vi "Parse Set Input.vi"(7 "error in (no error)":errorcluster caption="에러 입력(에러 없음)", 9 "JSON string":string, 10 "Instrument Manager 입력":refnum<class "Instrument Manager.lvclass">) -> (0 "error out":errorcluster caption="에러 출력", 1 "Input path":T1, 2 "Set Input Param":T2, 3 "Instrument Manager 출력":refnum<class "Instrument Manager.lvclass">)   [LabVIEW 2023, in "Instrument Manager.lvclass"]
uses:
  Instrument Manager.lvclass
  Param Definition/Set Input Path Param.ctl
  Instrument Manager.lvclass/Instrument Manager.ctl
  Module/CE RF Switch Box/Type Definition/Input path.ctl
  Module/CE RF Switch Box/RF Switch Box.lvlib
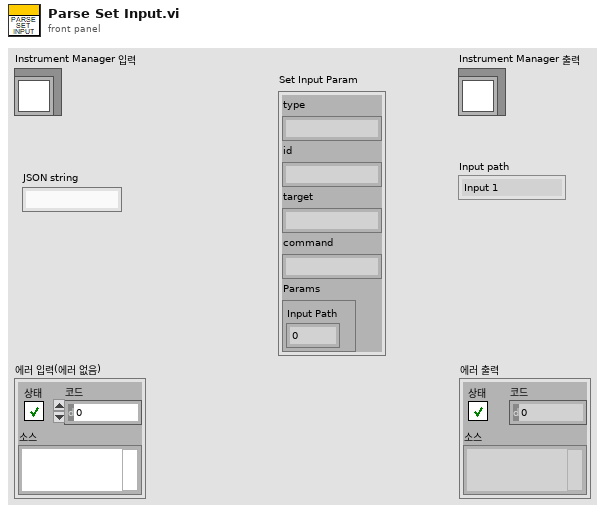
[diagram p1: front panel]
types:
  T1 = typedef "RF Switch Box.lvlib/Input path.ctl" = enum16{"Input 1", "Input 2", "Input 3"}
  T2 = typedef "Instrument Manager.lvclass/Set Input Path Param.ctl" = cluster{"type":string, "id":string, "target":string, "command":string, "Params":cluster{"Input Path":i32}}
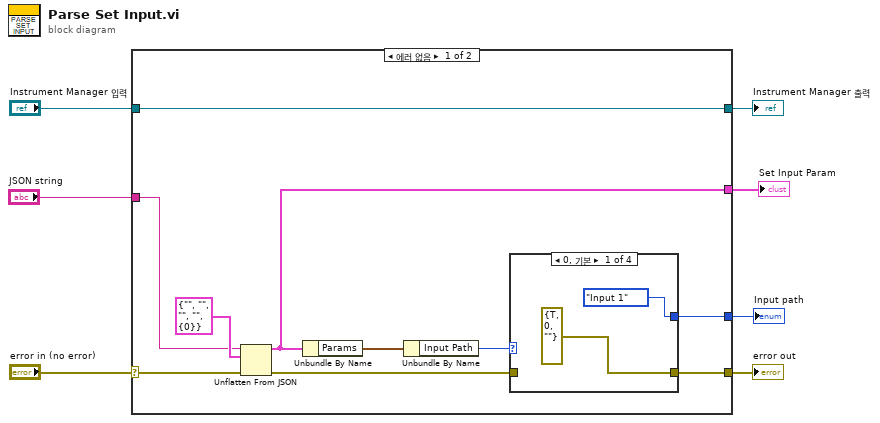
[diagram p0: block diagram]
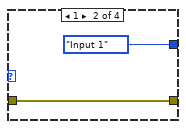
[diagram p2: hidden frame]
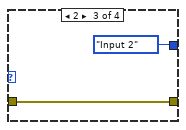
[diagram p3: hidden frame]
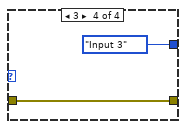
[diagram p4: hidden frame]
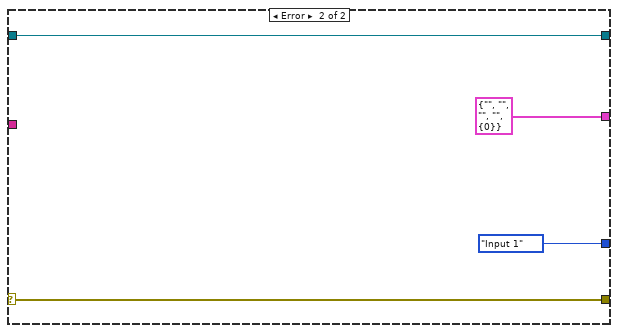
[diagram p5: hidden frame]
diagram:
  n1 = case shown="에러 없음" "error in (no error)" {
    selector: "error in (no error)" -> [w14 w29]
    tunnel: [w10 w29] -> w6
    tunnel: [w17 w28] -> w4
    tunnel: "Instrument Manager 입력" -> [w17 w28]
    tunnel: "JSON string" -> [w15 _]
    tunnel: [w9 T2 {"type"="", "id"="", "target"="", "command"="", "Params"={"Input Path"=0}} ("Set Input Param")] -> w2
    tunnel: [w8 Input_path."Input 1" ("Input path")] -> w1
    frame No Error {
      n2 = Unflatten From JSON(JSON string=w15, type and defaults=T2 {"type"="", "id"="", "target"="", "command"="", "Params"={"Input Path"=0}} ("Set Input Param"), error in (no error)=w14) -> (value=w9:T2, error out=w11:errorcluster)  [unwired: 4 in]
      n3 = Unbundle By Name(w9) -> ("Params"=w13:cluster{"Input Path":i32})
      n4 = Unbundle By Name(w13) -> ("Input Path"=w12:i32)
      n5 = case shown="0, 기본" w12 {
        tunnel: w11 -> [_ w21 w22 w24]
        tunnel: [errorcluster {"status"=TRUE, "code"=0, "source"=""} ("error out") w21 w22 w24] -> w10
        tunnel: [Input_path."Input 1" ("Input path") Input_path."Input 1" ("Input path") Input_path."Input 2" ("Input path") Input_path."Input 3" ("Input path")] -> w8
        frame 0, Default {
        }
        frame 1 {
        }
        frame 2 {
        }
        frame 3 {
        }
      }
    }
    frame Error {
    }
  }
  "error out" <- w6
  "Instrument Manager 출력" <- w4
  "Input path" <- w1
  "Set Input Param" <- w2
